vi "Open FPGA Ref.vi"(8 "error in (no error)":errorcluster, 10 "Bitfile Path":path, 11 "Device address":string) -> (0 "error out":errorcluster, 3 "FPGA Ref out":refnum<k20>)   [LabVIEW 2025, in "I2C Bus Monitor.lvclass"]
uses:
  I2C Bus Monitor.lvclass
  <vilib>/FPGAPlugInAG/Dynamic/niLvFpga_Close_Dynamic.vi
  Error Global.vi
  <vilib>/rvi/interface/nirviCloseFPGA/nirviCloseFPGA.xnode
  I2C Bus Monitor.lvclass/I2C Bus Monitor.ctl
  <instrlib>/FlexRIO/API/Host/v1/NI FlexRIO API v1.lvlib
  I2C Bus Monitor UI/I2C Bus Monitor UI.lvlib
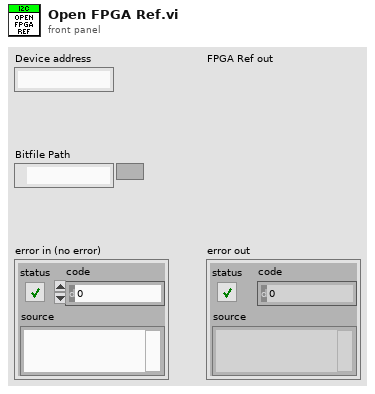
[diagram p1: front panel]
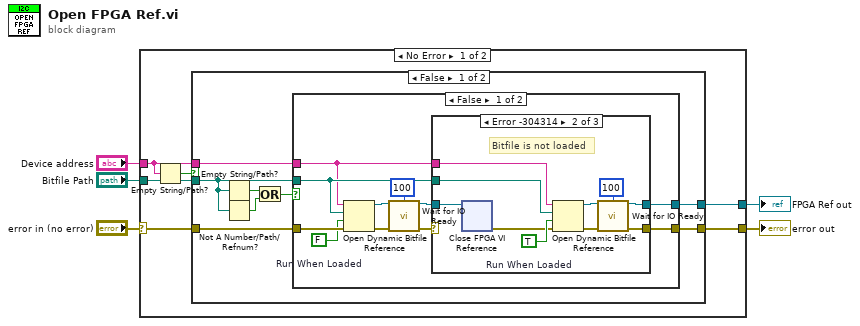
[diagram p0: block diagram]
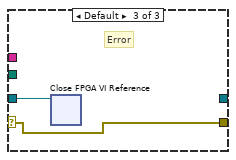
[diagram p3: hidden frame]
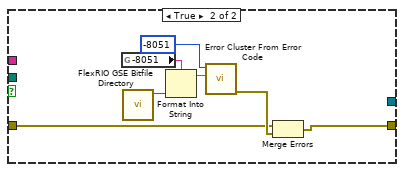
[diagram p4: hidden frame]
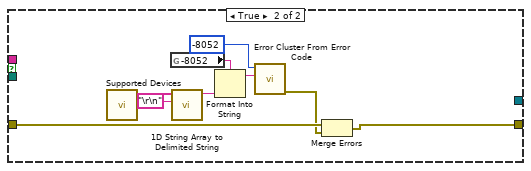
[diagram p5: hidden frame]
diagram:
  n1 = case shown="No Error" "error in (no error)" {
    selector: "error in (no error)" -> [w9 w61]
    tunnel: [w11 _] -> w5
    tunnel: [w10 w61] -> w4
    tunnel: "Bitfile Path" -> [w8 _]
    tunnel: "Device address" -> [w6 _]
    frame No Error {
      n2 = Empty String/Path?(string/path=w6) -> (empty?=w7:bool)
      n3 = case shown="False" w7 {
        tunnel: [w19 _] -> w11
        tunnel: [w18 w56] -> w10
        tunnel: w8 -> [w13 _]
        tunnel: w6 -> [w17 _]
        tunnel: w9 -> [w16 w57]
        frame False {
          n4 = Empty String/Path?(string/path=w13) -> (empty?=w14:bool)
          n5 = Not A Number/Path/Refnum?(number/path/refnum=w13) -> (NaN/Path/Refnum?=w15:bool)
          n6 = Or(x=w14, y=w15) -> (x .or. y?=w12:bool)
          n7 = case shown="False" w12 {
            tunnel: [w30 _] -> w19
            tunnel: [w29 w46] -> w18
            tunnel: w13 -> [w28 _]
            tunnel: w17 -> [w27 _]
            tunnel: w16 -> [w24 w47]
            frame False {
              w23 = FALSE  # Run When Loaded
              n8 = Open Dynamic Bitfile Reference(0:w27, 1:w28, 2:w23, 3:w24) -> (5:w21:refnum<k20>, 8:w22:errorcluster)  [unwired: 1 in]
              n9 = call <instrlib>:"Wait for IO Ready.vi"("fpga interface in"=w21, "timeout"=100, "error in"=w22) -> ("fpga interface out"=w26:refnum<k20>, "error out"=w25:errorcluster)  [unwired: 9 in, 2 out]
              n10 = case shown="Error -304314" w25 {
                selector: w25 -> [w32 _ w43]
                tunnel: [w32 w34 w43] -> w29
                tunnel: w26 -> [w31 w42 w44]
                tunnel: w27 -> [_ w36 _]
                tunnel: w28 -> [_ w35 _]
                tunnel: [w31 w33 _] -> w30
                frame No Error {
                  # "Bitfile is loaded"
                }
                frame Error {
                  w38 = TRUE  # Run When Loaded
                  # "Bitfile is not loaded"
                  n11 = xnode ("Close FPGA VI Reference")("FPGA VI Reference In"=w42) -> ("error out"=w37:errorcluster)  [unwired: 1 in]
                  n12 = Open Dynamic Bitfile Reference(0:w36, 1:w35, 2:w38, 3:w37) -> (5:w40:refnum<k20>, 8:w39:errorcluster)  [unwired: 1 in]
                  n13 = call <instrlib>:"Wait for IO Ready.vi"("fpga interface in"=w40, "timeout"=100, "error in"=w39) -> ("fpga interface out"=w33:refnum<k20>, "error out"=w34:errorcluster)  [unwired: 9 in, 2 out]
                }
                frame Default {
                  # "Error"
                  n14 = xnode ("Close FPGA VI Reference")("FPGA VI Reference In"=w44) -> ()  [unwired: 1 in, 1 out]
                }
              }
            }
            frame True {
              n15 = global read "Error Global.vi" "-8051"() -> (w51:string)
              n16 = call "FlexRIO GSE Bitfile Directory.vi"() -> ("Flexrio GSE Template Bitfiles Folder Path"=w45:path)  [unwired: 11 in]
              n17 = Format Into String(format string=w51, w45) -> (resulting string=w50:string)  [unwired: 2 in, 1 out]
              n18 = call <vilib>:"Error Cluster From Error Code.vi"("error message (\"\")"=w50, "error code (0)"=-8051) -> ("error out"=w48:errorcluster)  [unwired: 7 in]
              n19 = Merge Errors(w47, w48) -> (w46:errorcluster)
            }
          }
        }
        frame True {
          n20 = call "Supported Devices.vi"() -> ("Supported Devices"=w53:string[])  [unwired: 11 in]
          n21 = global read "Error Global.vi" "-8052"() -> (w60:string)
          n22 = call <vilib>:"1D String Array to Delimited String.vi"("delimiter"="\r\n", "string array"=w53) -> ("delimited string"=w52:string)  [unwired: 9 in]
          n23 = Format Into String(format string=w60, w52) -> (resulting string=w59:string)  [unwired: 2 in, 1 out]
          n24 = call <vilib>:"Error Cluster From Error Code.vi"("error message (\"\")"=w59, "error code (0)"=-8052) -> ("error out"=w55:errorcluster)  [unwired: 7 in]
          n25 = Merge Errors(w57, w55) -> (w56:errorcluster)
        }
      }
    }
    frame Error {
    }
  }
  "FPGA Ref out" <- w5
  "error out" <- w4
